vi "PixyCam_Loop.vi"(4 "error in":errorcluster, 6 "stop":bool, 7 "PixyCamDevRef":T1) -> (0 "error out":errorcluster, 3 "PixyCamDevRef Out":T1)   [LabVIEW 2016, in "PixyCam_LabVIEW.lvlib"]
uses:
  PixyCam_LabVIEW.lvlib
  Private/PixyCam_DevRef.ctl
  Private/PixyCam_SPI_DevRef.ctl
  <vilib>/Rock Robotics/WPI/SPI/WPI_SPIDevRef.ctl
  <vilib>/Rock Robotics/SystemInterfaces/spilib/spi_bus.ctl
  Private/PixyCam_CommMode.ctl
  Private/PixyCam_TargetData.ctl
  <vilib>/Utility/SystemLogging/NI_SystemLogging.lvlib
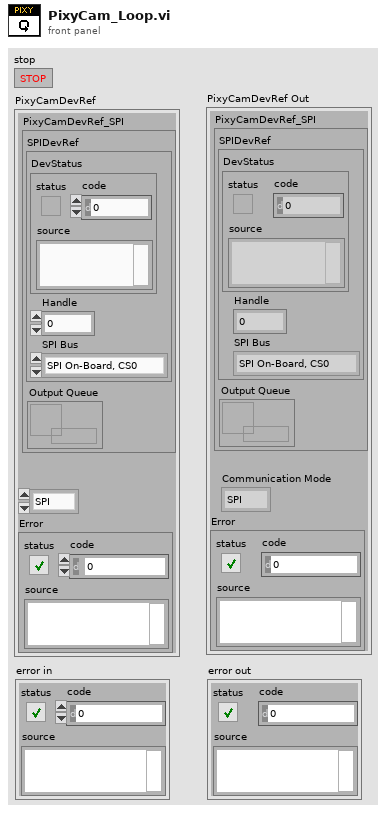
[diagram p1: front panel]
types:
  T1 = typedef "PixyCam_LabVIEW.lvlib/PixyCam_DevRef.ctl" = cluster{"PixyCamDevRef_SPI":T2, "Communication Mode":T5, "Error":errorcluster}
  T2 = typedef "PixyCam_LabVIEW.lvlib/PixyCam_SPI_DevRef.ctl" = cluster{"SPIDevRef":T3, "Output Queue":refnum<queue>}
  T3 = typedef "WPI_SPIDevRef.ctl" = cluster{"DevStatus":errorcluster, "Handle":i32, "SPI Bus":T4}
  T4 = typedef "spi_bus.ctl" = enum16{"SPI On-Board, CS0", "SPI On-Board, CS1", "SPI On-Board, CS2", "SPI On-Board, CS3", "SPI MXP", "Invalid"}
  T5 = typedef "PixyCam_LabVIEW.lvlib/PixyCam_CommMode.ctl" = enum16{"SPI", "I2C", "UART", "Analog", "Digital"}
  T6 = typedef "PixyCam_LabVIEW.lvlib/PixyCam_TargetData.ctl" = cluster{"Target Type":u16, "Checksum":u16, "Signature Number":u16, "X Center":u16, "Y Center":u16, "Width":u16, "Height":u16, "Angle":u16}
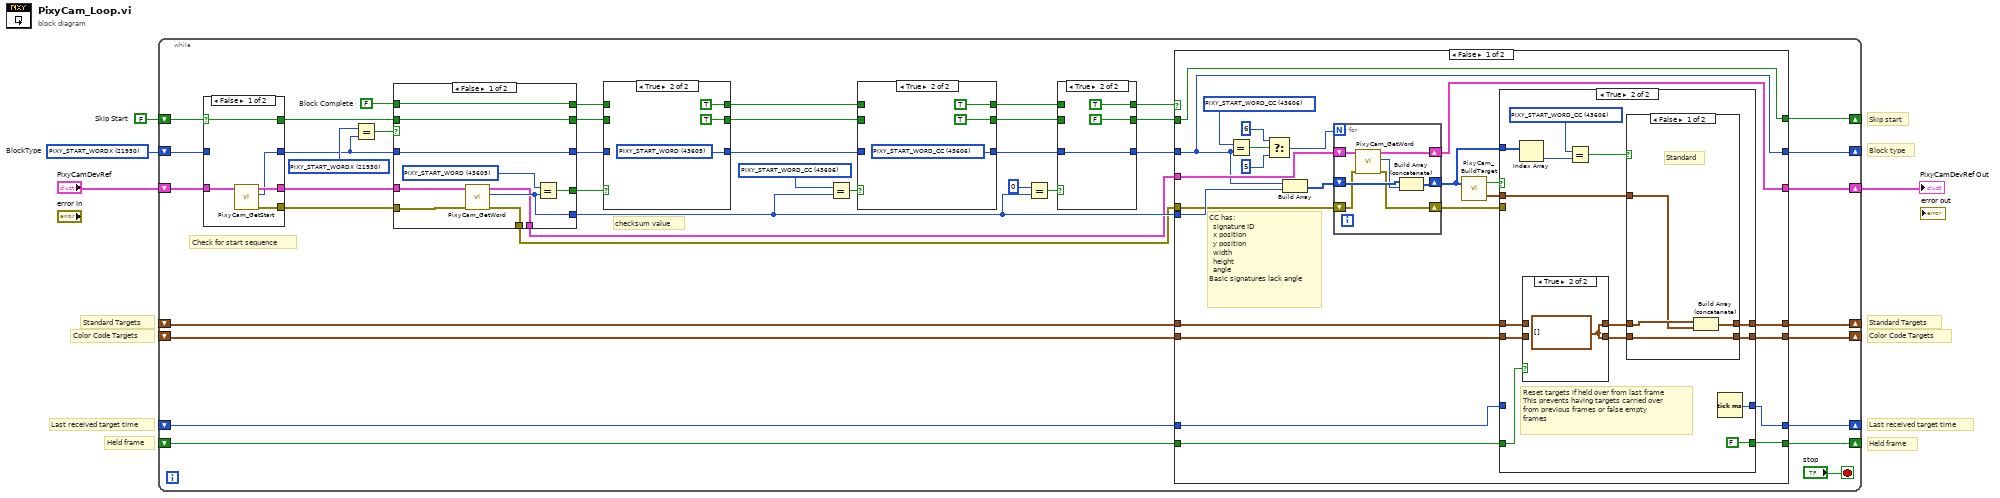
[diagram p0: block diagram]
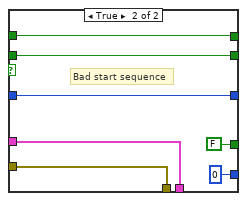
[diagram p2: hidden frame]
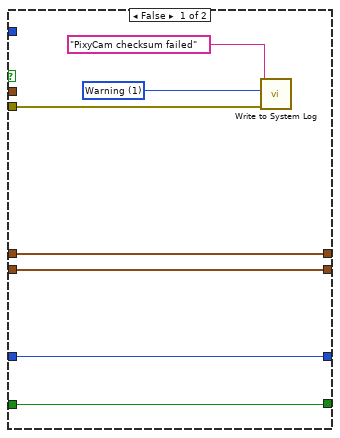
[diagram p3: hidden frame]
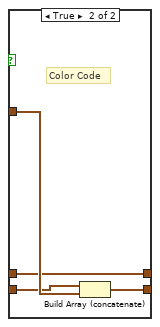
[diagram p5: hidden frame]
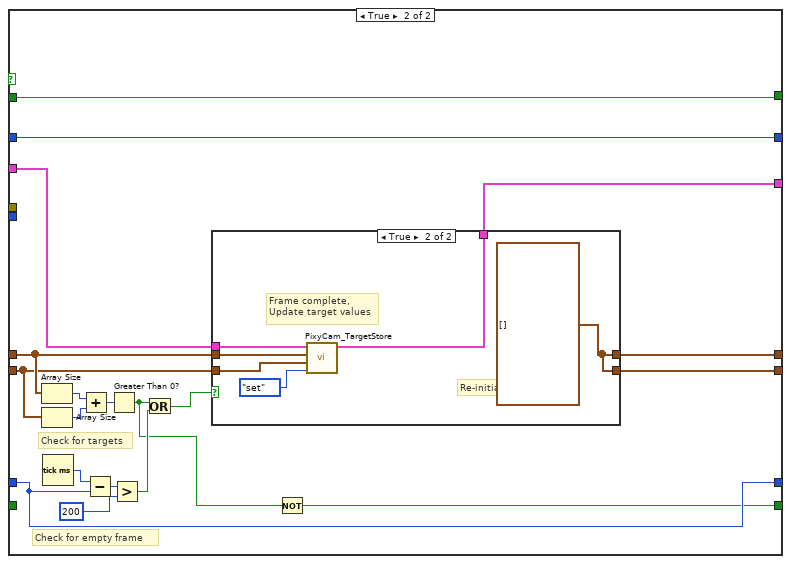
[diagram p6: hidden frame]
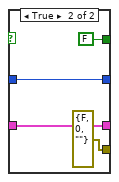
[diagram p11: hidden frame]
diagram:
  w1 = u16 21930 items=["PIXY_START_WORD"=43605, "PIXY_START_WORD_CC"=43606, "PIXY_START_WORDX"=21930]  # BlockType
  w2 = FALSE  # Skip Start
  # "Held frame"
  # "Held frame"
  # "Last received target time"
  # "Color Code Targets"
  # "Standard Targets"
  # "Last received target time"
  # "Color Code Targets"
  # "Standard Targets"
  # "Last received target time"
  # "Color Code Targets"
  # "Standard Targets"
  # "Last received target time"
  # "Color Code Targets"
  # "Standard Targets"
  # "Last received target time"
  # "Color Code Targets"
  # "Standard Targets"
  # "Last received target time"
  # "Color Code Targets"
  # "Standard Targets"
  # "Last received target time"
  # "Color Code Targets"
  # "Standard Targets"
  # "Last received target time"
  # "Color Code Targets"
  # "Standard Targets"
  # "Last received target time"
  # "Color Code Targets"
  # "Standard Targets"
  # "Last received target time"
  # "Color Code Targets"
  # "Standard Targets"
  # "Last received target time"
  # "Color Code Targets"
  # "Standard Targets"
  # "Last received target time"
  # "Color Code Targets"
  # "Standard Targets"
  # "Last received target time"
  # "Color Code Targets"
  # "Standard Targets"
  # "Last received target time"
  # "Color Code Targets"
  # "Standard Targets"
  # "Last received target time"
  # "Color Code Targets"
  # "Standard Targets"
  # "Last received target time"
  # "Color Code Targets"
  # "Standard Targets"
  # "Last received target time"
  # "Color Code Targets"
  # "Standard Targets"
  # "Last received target time"
  # "Color Code Targets"
  # "Standard Targets"
  # "Last received target time"
  # "Color Code Targets"
  # "Standard Targets"
  # "Last received target time"
  # "Color Code Targets"
  # "Standard Targets"
  # "Last received target time"
  # "Color Code Targets"
  # "Standard Targets"
  # "Last received target time"
  # "Color Code Targets"
  # "Standard Targets"
  # "Last received target time"
  # "Color Code Targets"
  # "Standard Targets"
  # "Last received target time"
  # "Color Code Targets"
  # "Standard Targets"
  # "Last received target time"
  # "Color Code Targets"
  # "Standard Targets"
  # "Last received target time"
  # "Color Code Targets"
  # "Standard Targets"
  # "Last received target time"
  # "Color Code Targets"
  # "Standard Targets"
  # "Last received target time"
  # "Color Code Targets"
  # "Standard Targets"
  # "Last received target time"
  # "Color Code Targets"
  # "Standard Targets"
  # "Last received target time"
  # "Color Code Targets"
  # "Standard Targets"
  # "Last received target time"
  # "Color Code Targets"
  # "Standard Targets"
  # "Last received target time"
  # "Color Code Targets"
  # "Standard Targets"
  # "Last received target time"
  # "Color Code Targets"
  # "Standard Targets"
  # "Last received target time"
  # "Color Code Targets"
  # "Standard Targets"
  # "Last received target time"
  # "Color Code Targets"
  # "Standard Targets"
  # "Last received target time"
  # "Color Code Targets"
  # "Standard Targets"
  # "Block type"
  # "Skip start"
  # "Last received target time"
  # "Color Code Targets"
  # "Standard Targets"
  n1 = while {
    shift-right: [w21] -> w3
    shift-left: "PixyCamDevRef" -> [w45]
    shift-right: [w24] -> _
    shift-left: w1 -> [w42]
    shift-right: [w22] -> _
    shift-left: w2 -> [w18]
    shift-right: [w28] -> _
    shift-left: _ -> [w25]
    shift-right: [w27] -> _
    shift-left: _ -> [w26]
    shift-right: [w20] -> _
    shift-left: _ -> [w19]
    shift-right: [w14] -> _
    shift-left: _ -> [w13]
    stop <- "stop" stop-if-true
    w11 = u16 21930 items=["PIXY_START_WORD"=43605, "PIXY_START_WORD_CC"=43606, "PIXY_START_WORDX"=21930] ("IDWord")
    w6 = FALSE  # Block Complete
    w39 = u16 43606 items=["PIXY_START_WORD"=43605, "PIXY_START_WORD_CC"=43606, "PIXY_START_WORDX"=21930] ("IDWord")
    # "checksum value"
    # "Check for start sequence"
    n2 = case shown="False" w18 {
      selector: w18 -> [w173 _]
      tunnel: w45 -> [w177 w181]
      tunnel: [w176 w181] -> w43
      tunnel: [w175 errorcluster {"status"=FALSE, "code"=0, "source"=""} ("error out")] -> w44
      tunnel: w42 -> [_ w180]
      tunnel: [w174 w180] -> w10
      tunnel: [w173 FALSE] -> w8
      frame False {
        n3 = call "PixyCam_GetStart.vi"("PixyCamDevRef"=w177) -> ("error out"=w175:errorcluster, "WordType"=w174:u16, "PixyCamDevRef Out"=w176:T1)  [unwired: 4 in]
      }
      frame True {
      }
    }
    n4 = Equal?(x=w11, y=w10) -> (x = y?=w12:bool)
    n5 = case shown="False" w12 {
      tunnel: w44 -> [w56 w62]
      tunnel: w43 -> [w55 w63]
      tunnel: [w53 u16 0 ("Word Out")] -> w32
      tunnel: [w52 w63] -> w30
      tunnel: [w51 w62] -> w29
      tunnel: [w50 FALSE] -> w17
      tunnel: w10 -> [w49 w59]
      tunnel: [w49 w59] -> w9
      tunnel: [w48 w57] -> w7
      tunnel: w8 -> [w48 w57]
      tunnel: [w47 w58] -> w5
      tunnel: w6 -> [w47 w58]
      frame False {
        w54 = u16 43605 items=["PIXY_START_WORD"=43605, "PIXY_START_WORD_CC"=43606, "PIXY_START_WORDX"=21930] ("IDWord")
        n6 = call "PixyCam_GetWord.vi"("error in"=w56, "PixyCamDevRef"=w55) -> ("error out"=w51:errorcluster, "Word Out"=w53:u16, "PixyCamDevRefOut"=w52:T1)  [unwired: 3 in]
        n7 = Equal?(x=w54, y=w53) -> (x = y?=w50:bool)
      }
      frame True {
        # "Bad start sequence"
      }
    }
    n8 = case shown="True" w17 {
      tunnel: w9 -> [w169 _]
      tunnel: [w169 w171] -> w40
      tunnel: [w168 TRUE] -> w41
      tunnel: w7 -> [w168 _]
      tunnel: [w167 TRUE] -> w38
      tunnel: w5 -> [w167 _]
      frame False {
      }
      frame True {
        w171 = u16 43605 items=["PIXY_START_WORD"=43605, "PIXY_START_WORD_CC"=43606, "PIXY_START_WORDX"=21930] ("IDWord")
      }
    }
    n9 = Equal?(x=w39, y=w32) -> (x = y?=w16:bool)
    n10 = case shown="True" w16 {
      tunnel: w40 -> [w163 _]
      tunnel: [w163 w165] -> w35
      tunnel: [w162 TRUE] -> w36
      tunnel: w41 -> [w162 _]
      tunnel: w38 -> [w161 _]
      tunnel: [w161 TRUE ("Block Complete")] -> w37
      frame False {
      }
      frame True {
        w165 = u16 43606 items=["PIXY_START_WORD"=43605, "PIXY_START_WORD_CC"=43606, "PIXY_START_WORDX"=21930] ("IDWord")
      }
    }
    n11 = Equal?(x=u16 0, y=w32) -> (x = y?=w15:bool)
    n12 = case shown="True" w15 {
      tunnel: w35 -> [w157 w158]
      tunnel: [w157 w158] -> w31
      tunnel: [w156 FALSE] -> w23
      tunnel: w36 -> [w156 _]
      tunnel: w37 -> [w155 _]
      tunnel: [w155 TRUE ("Block Complete")] -> w33
      frame False {
      }
      frame True {
      }
    }
    n13 = case shown="False" w33 {
      tunnel: w32 -> [w80 _]
      tunnel: w31 -> [w69 w143]
      tunnel: w30 -> [w81 w144]
      tunnel: w29 -> [w79 _]
      tunnel: [w75 w140] -> w28
      tunnel: [w73 w145] -> w27
      tunnel: w26 -> [w72 w139]
      tunnel: w25 -> [w71 w138]
      tunnel: [w69 w143] -> w24
      tunnel: [w70 w142] -> w22
      tunnel: w23 -> [w70 w142]
      tunnel: [w68 w141] -> w21
      tunnel: [w67 w129] -> w20
      tunnel: w19 -> [w66 w129]
      tunnel: [w65 w127] -> w14
      tunnel: w13 -> [w64 _]
      frame False {
        w87 = u16 43606 items=["PIXY_START_WORD"=43605, "PIXY_START_WORD_CC"=43606, "PIXY_START_WORDX"=21930] ("IDWord")
        # "CC has:\n  signature ID\n  x position\n  y position\n  width\n  height\n  angle\nBasic signatures lack angle"
        n14 = Equal?(x=w87, y=w69) -> (x = y?=w86:bool)
        n15 = Select(t=6, s=w86, f=5) -> (s? t:f=w83:i32)
        n16 = Build Array(w69, w80) -> (w82:u16[])
        n17 = for {
          N: w83 -> [_]
          shift-right: [w123] -> w74
          shift-left: w82 -> [w125]
          shift-right: [w122] -> w77
          shift-left: w79 -> [w121]
          shift-right: [w120] -> w68
          shift-left: w81 -> [w126]
          n18 = call "PixyCam_GetWord.vi"("error in"=w121, "PixyCamDevRef"=w126) -> ("error out"=w122:errorcluster, "Word Out"=w124:u16, "PixyCamDevRefOut"=w120:T1)  [unwired: 3 in]
          n19 = Build Array (concatenate)(w125, w124) -> (w123:u16[])
        }
        n20 = call "PixyCam_BuildTarget.vi"("RawData"=w74) -> ("Target"=w76:T6, "Valid Checksum"=w78:bool)  [unwired: 1 in]
        n21 = case shown="True" w78 {
          tunnel: w77 -> [w94 _]
          tunnel: w76 -> [_ w104]
          tunnel: [w90 w103] -> w75
          tunnel: w74 -> [_ w108]
          tunnel: [w91 w102] -> w73
          tunnel: w72 -> [w91 w96]
          tunnel: w71 -> [w90 w99]
          tunnel: [w89 w101] -> w67
          tunnel: w66 -> [w89 _]
          tunnel: [w88 FALSE] -> w65
          tunnel: w64 -> [w88 w95]
          frame False {
            w93 = 1 items=["Error", "Warning", "Informational"] ("severity")
            n22 = call <vilib>:"Write to System Log.vi"("error in (no error)"=w94, "severity"=w93, "message"="PixyCam checksum failed") -> ()  [unwired: 8 in, 1 out]
          }
          frame True {
            w106 = u16 43606 items=["PIXY_START_WORD"=43605, "PIXY_START_WORD_CC"=43606, "PIXY_START_WORDX"=21930] ("IDWord")
            # "Reset targets if held over from last frame\nThis prevents having targets carried over\nfrom previous frames or false empty\nframes"
            n23 = Index Array(array=w108) -> (element=w107:u16)  [unwired: 1 in]
            n24 = case shown="True" w95 {
              tunnel: w96 -> [w110 _]
              tunnel: w99 -> [w109 _]
              tunnel: [w110 w111] -> w98
              tunnel: [w109 w111] -> w97
              frame False {
              }
              frame True {
                w111 = T6[] []
              }
            }
            n25 = Equal?(x=w106, y=w107) -> (x = y?=w105:bool)
            n26 = case shown="False" w105 {
              tunnel: w104 -> [w113 w119]
              tunnel: [w112 w117] -> w103
              tunnel: [w114 w116] -> w102
              tunnel: w98 -> [w115 w116]
              tunnel: w97 -> [w112 w118]
              frame False {
                # "Standard"
                n27 = Build Array (concatenate)(w115, w113) -> (w114:T6[])
              }
              frame True {
                # "Color Code"
                n28 = Build Array (concatenate)(w118, w119) -> (w117:T6[])
              }
            }
            n29 = Tick Count (ms)() -> (millisecond timer value=w101:u32)
          }
        }
      }
      frame True {
        # "Check for targets"
        # "Check for empty frame"
        n30 = Array Size(array=w139) -> (size(s)=w137:i32)
        n31 = Array Size(array=w138) -> (size(s)=w136:i32)
        n32 = Tick Count (ms)() -> (millisecond timer value=w133:u32)
        n33 = Add(x=w137, y=w136) -> (x+y=w135:i32)
        n34 = Subtract(x=w133, y=w129) -> (x-y=w132:u32)
        n35 = Greater Than 0?(x=w135) -> (x > 0?=w128:bool)
        n36 = Greater?(x=w132, y=u32 200) -> (0:w130:bool)
        n37 = Or(x=w128, y=w130) -> (x .or. y?=w134:bool)
        n38 = case shown="True" w134 {
          tunnel: [w148 w149] -> w145
          tunnel: w144 -> [w146 w154]
          tunnel: w139 -> [w148 w153]
          tunnel: w138 -> [w147 w152]
          tunnel: [w146 w150] -> w141
          tunnel: [w147 w149] -> w140
          frame False {
          }
          frame True {
            w149 = T6[] []
            # "Re-initialize"
            # "Frame complete,\nUpdate target values"
            n39 = call "PixyCam_TargetStore.vi"("Operation"=enum16{"set", "get"}."set", "ColorCodeTargets Set"=w152, "StandardTargets Set"=w153, "PixyCamDevRef"=w154) -> ("PixyCamDevRef Out"=w150:T1)  [unwired: 1 in, 2 out]
          }
        }
        n40 = Not(x=w128) -> (.not. x?=w127:bool)
      }
    }
  }
  "PixyCamDevRef Out" <- w3
